vi "W07_Count_test.vi"() -> ()   [LabVIEW 2018]
doc: "Use this template to build a VI to use as a subVI."
panel:
  out "total[]":u32[](array[numeric])
  out "delta[]":u16[](array[numeric])
  out "raw[]":u16[](array[numeric])
  in  "fail[]":bool[](array[boolean])
  in  "value[] (D202 each second)":dbl[](array[numeric])
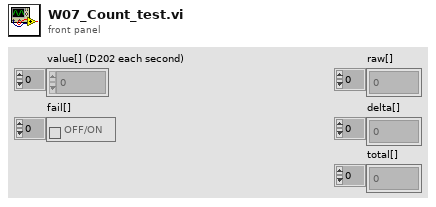
[diagram p1: front panel]
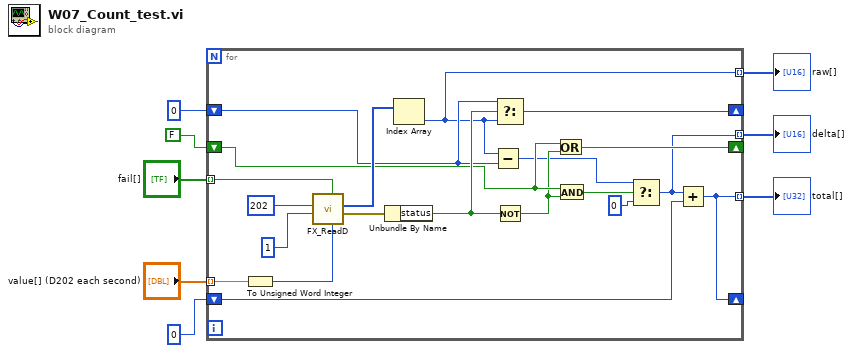
[diagram p0: block diagram]
diagram:
  n1 = for {
    tunnel: "value[] (D202 each second)" -> [w28] mode=indexing
    tunnel: "fail[]" -> [w26] mode=indexing
    shift-right: [w19] -> _
    shift-left: u16 0 ("value (sim)") -> [w20]
    shift-right: [w16] -> _
    shift-left: FALSE -> [w18]
    shift-right: [w9] -> _
    shift-left: u32 0 ("millisecond multiple") -> [w12]
    tunnel: [w11] -> w3 mode=indexing
    tunnel: [w10] -> w2 mode=indexing
    tunnel: [w9] -> w1 mode=indexing
    n2 = To Unsigned Word Integer(number=w28) -> (unsigned 16bit integer=w27:u16)
    n3 = call "FX_ReadD.vi"("value (sim)"=w27, "fail (sim)"=w26, "Count"=u16 1, "D"=u16 202) -> ("error out"=w22:errorcluster, "Words"=w23:u16[])  [unwired: 5 in, 1 out]
    n4 = Unbundle By Name(w22) -> ("status"=w21:bool)
    n5 = Index Array(array=w23) -> (element=w11:u16)  [unwired: 1 in]
    n6 = Subtract(x=w11, y=w20) -> (x-y=w14:u16)
    n7 = Select(t=w20, s=w21, f=w11) -> (s? t:f=w19:u16)
    n8 = Not(x=w21) -> (.not. x?=w17:bool)
    n9 = Or(x=w18, y=w17) -> (x .or. y?=w16:bool)
    n10 = And(x=w18, y=w17) -> (x .and. y?=w15:bool)
    n11 = Select(t=w14, s=w15, f=u16 0) -> (s? t:f=w10:u16)
    n12 = Add(x=w10, y=w12) -> (x+y=w9:u32)
  }
  "raw[]" <- w3
  "delta[]" <- w2
  "total[]" <- w1
